vi "CSM - Mark As Chain Module.vi"(6 "Order":i32, 9 "CSM Name":string="Chain") -> (2 "CSM Name (Marked As Chain)":string)   [LabVIEW 2017, in "Communicable State Machine.lvlib"]
doc: "Concatenates a Chain of Responsibility Mode module name using `$` as the separator. The order does not need to be consecutive, but it must be unique. Smaller numbers mean higher priority. During routing, CSM chooses the highest-priority node that can handle the message.\n\n<b>Reference Example</b>: `4. Advance Examples\\2. Chain of Responsibility Example`.\n\n\n> [!NOTE] <b>CSM Chain of Responsibility Mode</b>\n>\n> Multiple CSM modules form a Chain module by appending `$` and a number to the requested name.\n> - From an external call perspective, these instances collectively form a composite module named Chain.\n> - Each instance is named a Chain Node.\n>\n> <b>Behavior</b>: External callers can consider the Chain as a single CSM module capable of message communication, state registration, and so on. Internally, CSM uses the Chain registry to route a message directly to the highest-priority node that can handle it (smaller number = higher priority). A message is handled by only one node; it is not passed sequentially or downgraded across nodes.\n>\n> <b>Communication Restriction</b>: Messages must be sent to the Chain module name, not to a specific `ChainName$N` node.\n>\n> <b>Example</b>:\n>\n> // Request module name as `module$`, where `module` is the chain name. Instantiate 4 instances. Their names might be:\n> // - `module$1`\n> // - `module$2`\n> // - `module$3`\n> // - `module$4`\n> // Assume `module$3` and `module$4` can process \"csm message\"\n> `csm message >> arguments -@ module`\n> // CSM routes the message directly to the higher-priority `module$3`; `module$4` will not respond.\n>\n> <b>Application Scenarios</b>:\n> - Function composition: Different nodes handle different message types while exposing one Chain module externally.\n> - Function overriding: When multiple nodes implement the same message type, the higher-priority node takes effect.\n\n\n> [!NOTE] <b>Name Concatenation API</b>\n>\n> This VI only manipulates the module name string and has no actual functionality. Therefore, once you are familiar with the CSM rules, you can directly enter name string and rule symbols without calling this API.\n\n\n-- <b>Controls</b> --\n- <b>CSM Name</b>: CSM module name.\n- <b>Order</b>: Priority number in Chain of Responsibility Mode. Smaller numbers mean higher priority, and the value must be unique within the same Chain.\n\n-- <b>Indicators</b> --\n- <b>CSM Name (Marked As Chain)</b>: CSM module name marked with `$`."
uses:
  Communicable State Machine.lvlib
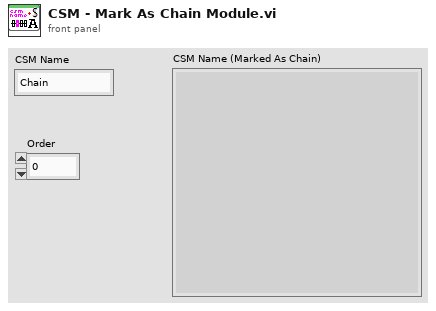
[diagram p1: front panel]
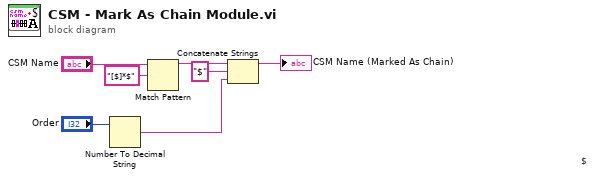
[diagram p0: block diagram]
diagram:
  # "$"
  n1 = Number To Decimal String(number="Order") -> (decimal integer string=w1:string)  [unwired: 1 in]
  n2 = Match Pattern(string="CSM Name", regular expression="[$]*$") -> (before substring=w5:string)  [unwired: 1 in, 3 out]
  n3 = Concatenate Strings(w5, "$" ("string"), w1) -> (→"CSM Name (Marked As Chain)":string)
